vi "case --- calculator.vi"() -> ()   [LabVIEW 2018]
panel:
  in  "condition":string
  out "Waveform Chart":dbl(graph)
  out "output":dbl
  in  "x":dbl
  in  "y":dbl
  # "CALCULATOR"
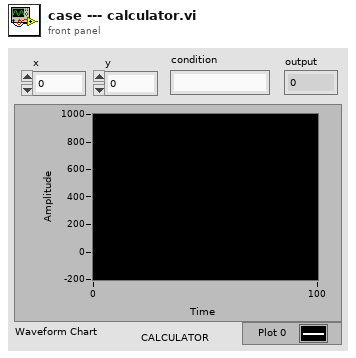
[diagram p1: front panel]
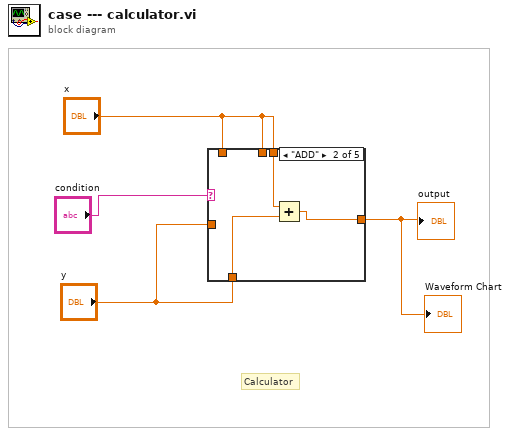
[diagram p0: block diagram]
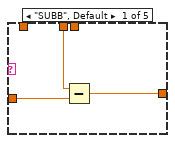
[diagram p2: hidden frame]
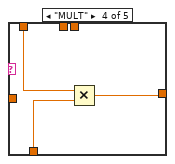
[diagram p4: hidden frame]
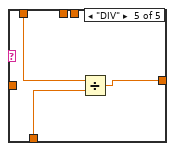
[diagram p5: hidden frame]
diagram:
  # "Calculator"
  n1 = case shown="\"ADD\"" "condition" {
    tunnel: "x" -> [_ w10 _ _ _]
    tunnel: "y" -> [_ w9 _ w12 w15]
    tunnel: "y" -> [w7 _ _ _ _]
    tunnel: "x" -> [w6 _ _ _ _]
    tunnel: "x" -> [_ _ _ w13 w16]
    tunnel: [w5 w8 _ w11 w14] -> w2
    frame "SUBB", Default {
      n2 = Subtract(x=w6, y=w7) -> (x-y=w5:dbl)
    }
    frame "ADD" {
      n3 = Add(x=w10, y=w9) -> (x+y=w8:dbl)
    }
    frame "EMPTY" {
      # "RIGHT CLICK\nUSE DEFAULT"
    }
    frame "MULT" {
      n4 = Multiply(x=w13, y=w12) -> (x*y=w11:dbl)
    }
    frame "DIV" {
      n5 = Divide(x=w16, y=w15) -> (x/y=w14:dbl)
    }
  }
  "output" <- w2
  "Waveform Chart" <- w2
